vi "Bridge_Loop.vi"(8 "error in (no error)":errorcluster={"status"=FALSE, "code"=0, "source"="\"\""}, 10 "ActivePlanRef":string="PLAN_01", 11 "IncomingCommand":string="CMD_START") -> (0 "error out":errorcluster={"status"=FALSE, "code"=0, "source"="\"\""}, 2 "status ok":bool, 3 "DispatchedResult":string)   [LabVIEW 2026]
doc: "INTENT: Hardware bridge command arbiter loop validating and dispatching setpoints."
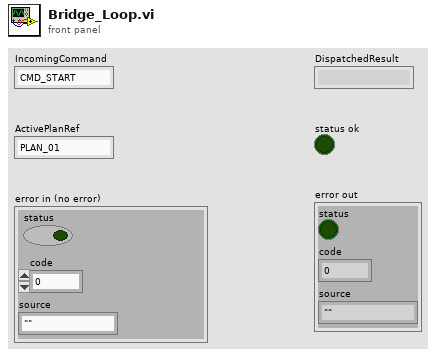
[diagram p1: front panel]
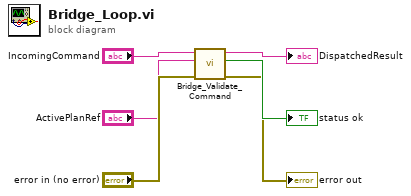
[diagram p0: block diagram]
diagram:
  n1 = call "Bridge_Validate_Command.vi"("error in (no error)"="error in (no error)", "active plan"="ActivePlanRef", "CommandRequest"="IncomingCommand") -> ("error out"=→"error out":errorcluster, "status ok"=→"status ok":bool, "Authorized/rejected reason"=→"DispatchedResult":string)  [unwired: 6 in]
